vi "Single DM Control.vi"(7 "Calling VI Ref":refnum<vi>) -> ()   [LabVIEW 2016]
uses:
  Controls/Pixel Scan Parameters.ctl
  Controls/MirrorModes.ctl
  <vilib>/Utility/miscctls.llb/LVPointTypeDef.ctl
  Hardware Configuration/Hardware Configuration Controls/Standard Action.ctl
  <vilib>/Analysis/baseanly.llb/Mean (DBL).vi
  <vilib>/Utility/file.llb/Write Delimited Spreadsheet (DBL).vi
  <vilib>/Utility/file.llb/Read Delimited Spreadsheet (DBL).vi
  <vilib>/Analysis/NI_AALBase.lvlib
panel:
  in  "Load Control Matrix":bool
  in  "Bias Level":dbl format="%#_13g"
  in  "Load Flat":bool
  in  "Apply Zero":bool
  in  "Load V Map":bool
  in  "Save V Map":bool
  in  "Apply Flat":bool
  in  "Center Bias":bool
  in  "Quit":bool
  in  "Mirror Tab":enum32{"Mirror Modes", "Scan Pixels", "Poke"}(tab)
  in  "Clear Modes":bool
  in  "Mirror Modes":T1
  in  "Load Modes":bool
  in  "Save Modes":bool
  in  "Scan Modes":bool
  in  "Pixel Scan Save Path":path
  in  "Save Data":bool
  in  "Pixel Scan Parameters":T2={"Scan Start Pixel"=1, "Scan End Pixel"=1, "Pixel Start Value (-1 to 1)"=-0.5, "Pixel End Value (-1 to 1)"=0.5, "Number of Steps"=0.1}
  in  "Start Pixel Scan":bool
  in  "Poke Amount":dbl=1.0
  in  "Pixel No.":i32=1
  in  "Poke":bool
  in  "Poke Unit":T3(radio)
  out "Pixel Map (-1 to 1)":dbl[][](graph)
  # "Mode"
  # "Amount (nm)"
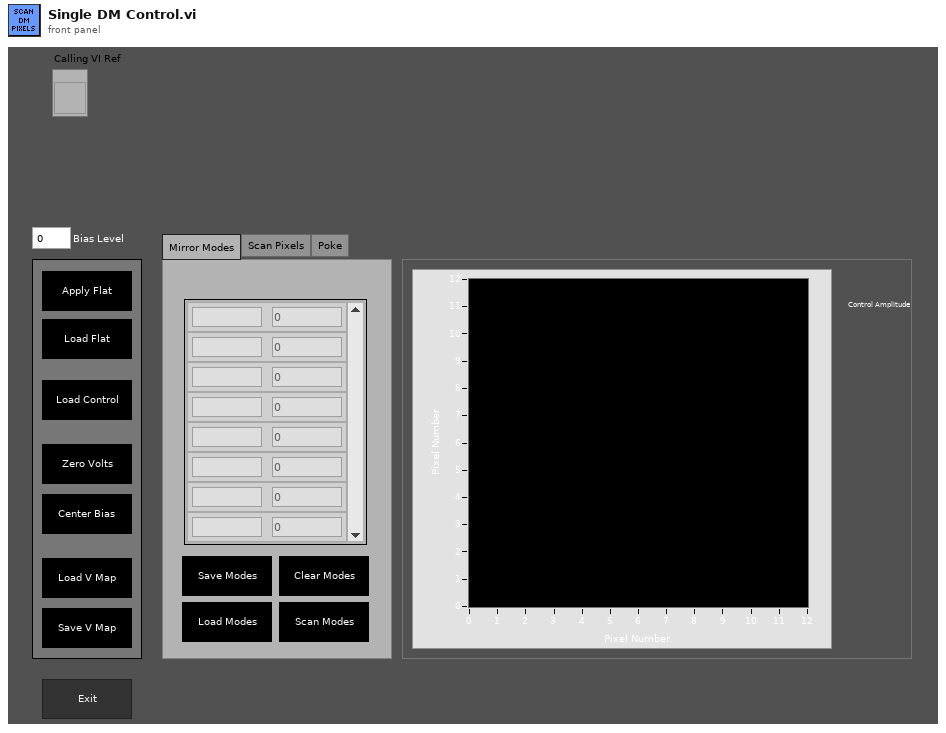
[diagram p1: front panel]
types:
  T1 = typedef "MirrorModes.ctl" = cluster{"Mode":string, "Amplitude":dbl}[]
  T2 = typedef "Pixel Scan Parameters.ctl" = cluster{"Scan Start Pixel":i32, "Scan End Pixel":i32, "Pixel Start Value (-1 to 1)":dbl, "Pixel End Value (-1 to 1)":dbl, "Number of Steps":dbl}
  T3 = enum32{"Voltage (V)", "Control Parameter [-1, 1]", "Approx. Distance (nm)"}
  T4 = enum16{"Always On", "Always Off", "Off While Running"}
  T5 = typedef "LVPointTypeDef.ctl" = cluster{"Horizontal":i16, "Vertical":i16}
  T6 = typedef "LVRectTypeDef.ctl" = cluster{"Left":i16, "Top":i16, "Right":i16, "Bottom":i16}
  T7 = typedef "LVBoundsTypeDef.ctl" = cluster{"Width":u32, "Height":u32}
  T8 = typedef "Standard Action.ctl" = enum16{"Read", "Write"}
  T9 = enum16{"Start Scan", "Reset Counter", "Write DM", "Get Image", "Update Count", "Exit"}
  T10 = enum32{"Invalid", "Standard", "Closed", "Hidden", "Minimized", "Maximized"}
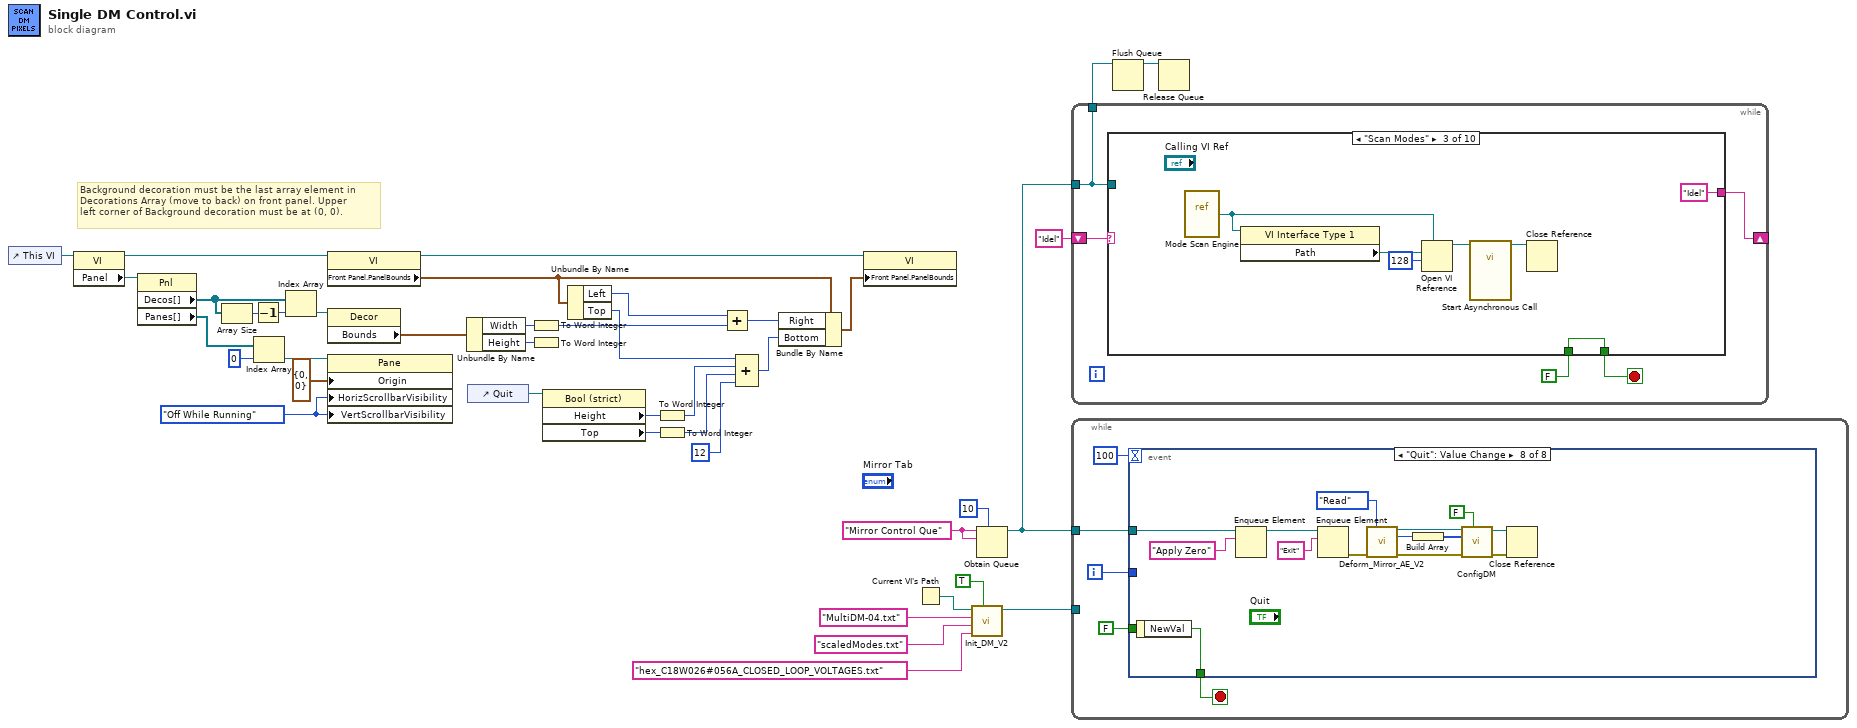
[diagram p0: block diagram]
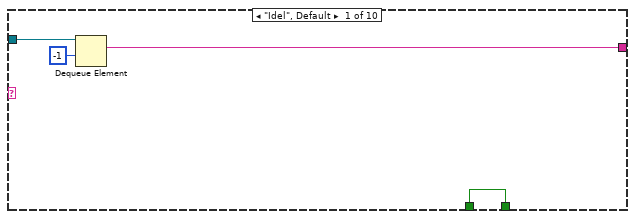
[diagram p2: hidden frame]
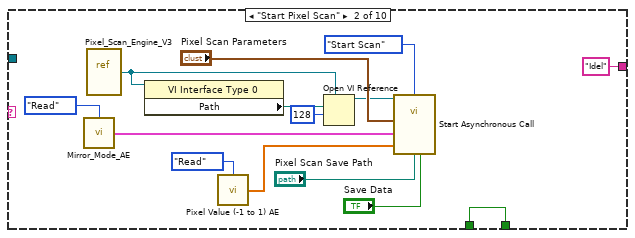
[diagram p3: hidden frame]
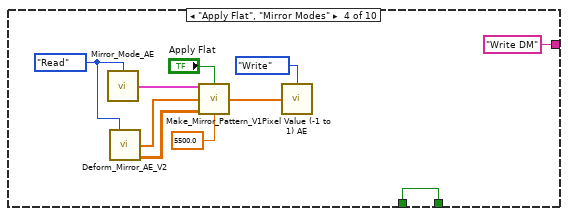
[diagram p4: hidden frame]
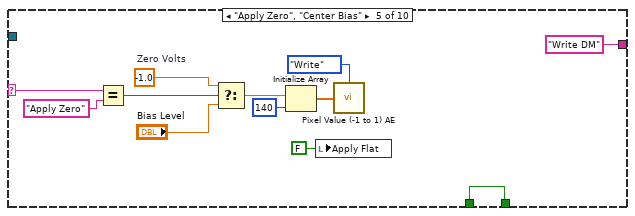
[diagram p5: hidden frame]
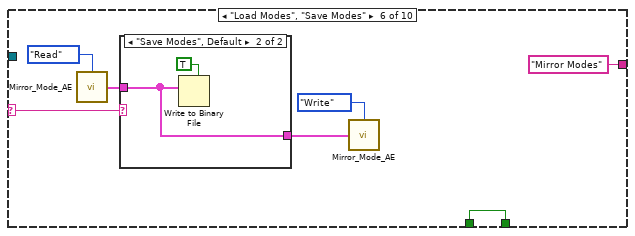
[diagram p6: hidden frame]
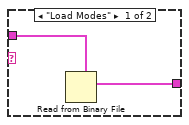
[diagram p7: hidden frame]
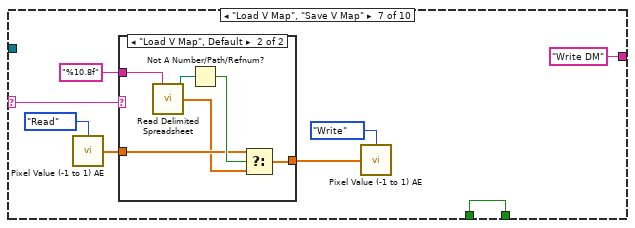
[diagram p8: hidden frame]
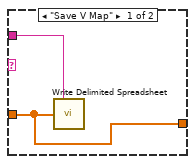
[diagram p9: hidden frame]
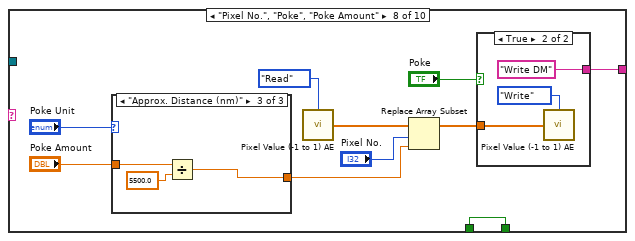
[diagram p10: hidden frame]
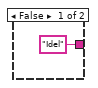
[diagram p11: hidden frame]
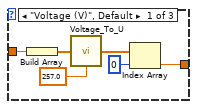
[diagram p12: hidden frame]
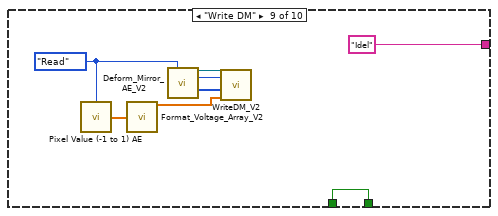
[diagram p14: hidden frame]
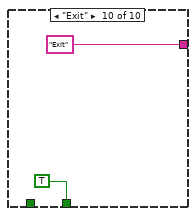
[diagram p15: hidden frame]
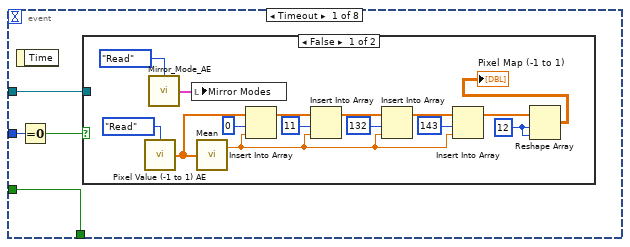
[diagram p16: hidden frame]
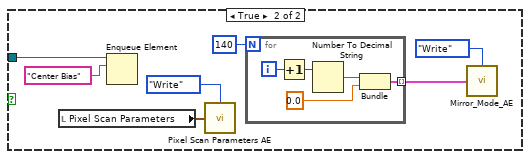
[diagram p17: hidden frame]
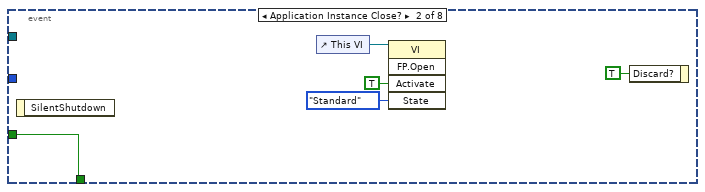
[diagram p18: hidden frame]
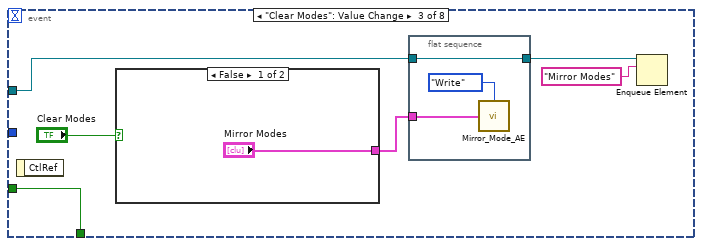
[diagram p19: hidden frame]
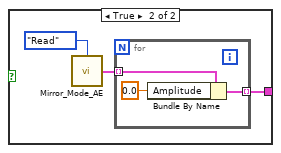
[diagram p20: hidden frame]
diagram:
  w12 = T4."Off While Running" ("Vertical Scrollbar Visibility")
  w41 = "Mirror Control Que" ("name (unnamed)")
  # "Background decoration must be the last array element in\nDecorations Array (move to back) on front panel. Upper\nleft corner of Background decoration must be at (0, 0)."
  n1 = control-ref of="This VI"() -> (w5:refnum<vi>)
  n2 = property class="VI"(reference=w5) -> (reference out=w13:refnum<vi>, "Panel"=w6:refnum<vi>)  [unwired: 1 in, 1 out]
  n3 = property class="Pnl"(reference=w6) -> ("Decos[]"=w4:refnum<vi>[], "Panes[]"=w9:refnum<vi>[])  [unwired: 1 in, 2 out]
  n4 = Array Size(array=w4) -> (size(s)=w2:i32)
  n5 = Decrement(x=w2) -> (x-1=w3:i32)
  n6 = Index Array(array=w9, index=0) -> (element=w8:refnum<vi>)
  n7 = Index Array(array=w4, index=w3) -> (element=w11:refnum<vi>)
  n8 = property class="VI"(reference=w13) -> (reference out=w15:refnum<vi>, "Front Panel.PanelBounds"=w16:T6)  [unwired: 1 in, 1 out]
  n9 = property class="Decor"(reference=w11) -> ("Bounds"=w14:T7)  [unwired: 1 in, 2 out]
  n10 = property class="Pane"(reference=w8, "Origin"=T5 {"Horizontal"=0, "Vertical"=0}, "HorizScrollbarVisibility"=w12, "VertScrollbarVisibility"=w12) -> ()  [unwired: 1 in, 2 out]
  n11 = Unbundle By Name(w14) -> ("Width"=w19:u32, "Height"=w22:u32)
  n12 = control-ref of="Quit"() -> (w1:refnum<vi>)
  n13 = To Word Integer(number=w19) -> (16bit integer=w21:i16)
  n14 = To Word Integer(number=w22) -> ()  [unwired: 1 out]
  n15 = property class="Bool (strict)"(reference=w1) -> ("Height"=w24:u32, "Top"=w25:i32)  [unwired: 1 in, 2 out]
  n16 = Unbundle By Name(w16) -> ("Left"=w18:i16, "Top"=w29:i16)
  n17 = To Word Integer(number=w24) -> (16bit integer=w27:i16)
  n18 = To Word Integer(number=w25) -> (16bit integer=w28:i16)
  n19 = Add(x=w18, y=w21) -> (x+y=w20:i16)
  n20 = Compound Arithmetic op=ADD(w29, w27, w28, i16 12 ("y")) -> (w23:i16)
  n21 = Bundle By Name(cluster=w16, "Right"=w20, "Bottom"=w23) -> (w17:T6)
  n22 = property class="VI"(reference=w15, "Front Panel.PanelBounds"=w17) -> ()  [unwired: 1 in, 2 out]
  n23 = Current VI's Path() -> (path=w33:path)
  n24 = call "Init_DM_V2.vi"("BM Flat"=TRUE, "BM Flat File"="hex_C18W026#056A_CLOSED_LOOP_VOLTAGES.txt" ("name or relative path"), "Mirror Modes File"="scaledModes.txt" ("name or relative path"), "DM Mapping File"="MultiDM-04.txt" ("name or relative path"), "Base File Path"=w33) -> ("reference out"=w39:refnum<k7>)  [unwired: 6 in]
  n25 = Obtain Queue(max queue size (-1, unlimited)=10, name (unnamed)=w41, element data type=w41) -> (queue out=w35:refnum<queue>)  [unwired: 2 in, 2 out]
  n26 = while {
    tunnel: w35 -> [w42]
    shift-right: [w46] -> _
    shift-left: "Idel" ("name (unnamed)") -> [w45]
    tunnel: [w42] -> w38
    stop <- w44 stop-if-true
    n27 = case shown="\"Scan Modes\"" w45 {
      selector: w45 -> [_ _ _ _ w88 w96 w111 _ _ _]
      tunnel: w42 -> [w50 _ _ _ _ _ _ _ _ _]
      tunnel: [w48 "Idel" ("name (unnamed)") "Idel" ("name (unnamed)") "Write DM" ("name (unnamed)") "Write DM" ("name (unnamed)") "Mirror Modes" ("name (unnamed)") "Write DM" ("name (unnamed)") w122 "Idel" ("name (unnamed)") "Exit" ("name (unnamed)")] -> w46
      tunnel: [w47 w64 w71 w80 w93 w100 w112 w130 w152 TRUE] -> w44
      tunnel: FALSE -> [w47 w64 w71 w80 w93 w100 w112 w130 w152 _]
      frame "Idel", Default {
        n28 = Dequeue Element(queue=w50, timeout in ms (-1)=-1) -> (element=w48:string)  [unwired: 1 in, 3 out]
      }
      frame "Start Pixel Scan" {
        n29 = call "Mirror_Mode_AE.vi"("Action"=Standard_Action."Read") -> ("Mirror Modes Out"=w51:T1)  [unwired: 14 in]
        n30 = vi-ref "Pixel_Scan_Engine_V3.vi"() -> (w55:refnum<vi>)
        n31 = property class="VI Interface Type 0"(reference=w55) -> ("Path"=w53:path)  [unwired: 1 in, 2 out]
        n32 = call "Pixel Value (-1 to 1) AE.vi"("Action"=Standard_Action."Read") -> ("Pixel Value (-1 to 1) Out"=w62:dbl[])  [unwired: 14 in]
        n33 = Open VI Reference(type specifier VI Refnum (for type only)=w55, vi path=w53, options=128) -> (vi reference=w56:refnum<vi>)  [unwired: 3 in, 1 out]
        n34 = call-by-ref "Start Asynchronous Call"(reference=w56, "Pixel Scan Parameters In"="Pixel Scan Parameters", "Action"=T9."Start Scan", "Initial Mirror Modes"=w51, "Initial Pixel Values (-1 to 1)"=w62, "Base Save Path"="Pixel Scan Save Path", "Save Data"="Save Data") -> ()  [unwired: 11 in, 2 out]
      }
      frame "Scan Modes" {
        n35 = vi-ref "Mode Scan Engine.vi"() -> (w65:refnum<vi>)
        n36 = property class="VI Interface Type 1"(reference=w65) -> ("Path"=w66:path)  [unwired: 1 in, 2 out]
        n37 = Open VI Reference(type specifier VI Refnum (for type only)=w65, vi path=w66, options=128) -> (vi reference=w68:refnum<vi>)  [unwired: 3 in, 1 out]
        n38 = call-by-ref "Start Asynchronous Call"(reference=w68) -> (reference out=w69:refnum<vi>)  [unwired: 17 in, 1 out]
        n39 = Close Reference(reference=w69) -> ()  [unwired: 1 in, 1 out]
      }
      frame "Apply Flat", "Mirror Modes" {
        w74 = Standard_Action."Read" ("Action")
        n40 = call "Mirror_Mode_AE.vi"("Action"=w74) -> ("Mirror Modes Out"=w77:T1)  [unwired: 14 in]
        n41 = call "Deform_Mirror_AE_V2.vi"("Action"=w74) -> ("Flat Files Out"=w78:dbl[], "Mode Matrix Out"=w79:dbl[][])  [unwired: 10 in, 3 out]
        n42 = call "Make_Mirror_Pattern_V1.vi"("Mirror Modes In"=w77, "Flat On?"="Apply Flat", "Flat File In"=w78, "Mirror Modes Array"=w79, "Amplitude Scale Factor"=5500.0) -> ("Pixel Value U (-1 to 1)"=w76:dbl[])  [unwired: 10 in]
        n43 = call "Pixel Value (-1 to 1) AE.vi"("Action"=Standard_Action."Write", "Pixel Value (-1 to 1)"=w76) -> ()  [unwired: 13 in, 1 out]
      }
      frame "Apply Zero", "Center Bias" {
        w84 = -1.0  # Zero Volts
        n44 = Equal?(x=w88, y="Apply Zero") -> (x = y?=w87:bool)
        n45 = Select(t=w84, s=w87, f="Bias Level") -> (s? t:f=w85:dbl)
        n46 = Initialize Array(w85, 140 ("dimension size")) -> (w91:dbl[])
        n47 = local write "Apply Flat"(FALSE ("Apply Flat")) -> ()
        n48 = call "Pixel Value (-1 to 1) AE.vi"("Action"=Standard_Action."Write", "Pixel Value (-1 to 1)"=w91) -> ()  [unwired: 13 in, 1 out]
      }
      frame "Load Modes", "Save Modes" {
        n49 = call "Mirror_Mode_AE.vi"("Action"=Standard_Action."Read") -> ("Mirror Modes Out"=w95:T1)  [unwired: 14 in]
        n50 = case shown="\"Save Modes\", Default" w96 {
          tunnel: w95 -> [w102 w103]
          tunnel: [w101 w103] -> w94
          frame "Load Modes" {
            n51 = Read from Binary File(5:w102) -> (2:w101:T1)  [unwired: 5 in, 3 out]
          }
          frame "Save Modes", Default {
            n52 = Write to Binary File(data=w103, 5:TRUE ("prepend array or string size? (T)")) -> ()  [unwired: 4 in, 3 out]
          }
        }
        n53 = call "Mirror_Mode_AE.vi"("Action"=Standard_Action."Write", "Mirror Modes In"=w94) -> ()  [unwired: 13 in, 1 out]
      }
      frame "Load V Map", "Save V Map" {
        n54 = call "Pixel Value (-1 to 1) AE.vi"("Action"=Standard_Action."Read") -> ("Pixel Value (-1 to 1) Out"=w109:dbl[])  [unwired: 14 in]
        n55 = case shown="\"Load V Map\", Default" w111 {
          tunnel: w109 -> [w113 w117]
          tunnel: "%10.8f" -> [w114 w120]
          tunnel: [w113 w115] -> w105
          frame "Save V Map" {
            n56 = call-poly <vilib>:"Write Delimited Spreadsheet.vi"("format (%.3f)"=w114, "1D data"=w113) -> ()  [unwired: 12 in, 2 out]
          }
          frame "Load V Map", Default {
            n57 = call-poly <vilib>:"Read Delimited Spreadsheet.vi"("format (%.3f)"=w120) -> ("new file path (Not A Path if cancelled)"=w119:path, "first row"=w116:dbl[])  [unwired: 9 in, 4 out]
            n58 = Not A Number/Path/Refnum?(number/path/refnum=w119) -> (NaN/Path/Refnum?=w118:bool)
            n59 = Select(t=w117, s=w118, f=w116) -> (s? t:f=w115:dbl[])
          }
        }
        n60 = call "Pixel Value (-1 to 1) AE.vi"("Action"=Standard_Action."Write", "Pixel Value (-1 to 1)"=w105) -> ()  [unwired: 13 in, 1 out]
      }
      frame "Pixel No.", "Poke", "Poke Amount" {
        n61 = case shown="\"Approx. Distance (nm)\"" "Poke Unit" {
          tunnel: "Poke Amount" -> [w139 w141 w144]
          tunnel: [w135 w141 w142] -> w128
          frame "Voltage (V)", Default {
            n62 = Build Array(w139) -> (w138:dbl[])
            n63 = call "Voltage_To_U.vi"("Voltages In (Volts)"=w138, "Mirror Max Voltage (Volts)"=257.0) -> ("Pixel Value (-1 to 1)"=w137:dbl[])  [unwired: 13 in]
            n64 = Index Array(array=w137, index=0) -> (element=w135:dbl)
          }
          frame "Control Parameter [-1, 1]" {
          }
          frame "Approx. Distance (nm)" {
            n65 = Divide(x=w144, y=5500.0) -> (x/y=w142:dbl)
          }
        }
        n66 = call "Pixel Value (-1 to 1) AE.vi"("Action"=Standard_Action."Read") -> ("Pixel Value (-1 to 1) Out"=w129:dbl[])  [unwired: 14 in]
        n67 = Replace Array Subset(array=w129, new element=w128, index="Pixel No.") -> (w123:dbl[])
        n68 = case shown="True" "Poke" {
          tunnel: w123 -> [_ w133]
          tunnel: ["Idel" ("name (unnamed)") "Write DM" ("name (unnamed)")] -> w122
          frame False {
          }
          frame True {
            n69 = call "Pixel Value (-1 to 1) AE.vi"("Action"=Standard_Action."Write", "Pixel Value (-1 to 1)"=w133) -> ()  [unwired: 13 in, 1 out]
          }
        }
      }
      frame "Write DM" {
        w150 = Standard_Action."Read" ("Action")
        n70 = call "Pixel Value (-1 to 1) AE.vi"("Action"=w150) -> ("Pixel Value (-1 to 1) Out"=w149:dbl[])  [unwired: 14 in]
        n71 = call "Format_Voltage_Array_V2.vi"("Pixel Level (-1 to 1)"=w149) -> ("Voltage Array (Volts)"=w145:dbl[])  [unwired: 13 in, 1 out]
        n72 = call "Deform_Mirror_AE_V2.vi"("Action"=w150) -> ("Refnum Out"=w148:refnum<k7>, "IDs Out"=w147:i32, "Multi Map Data Out"=w146:i32[])  [unwired: 10 in, 2 out]
        n73 = call "WriteDM_V2.vi"("reference in"=w148, "nDevId"=w147, "MultiDM  Mapping"=w146, "Voltage Array in"=w145) -> ()  [unwired: 2 in, 2 out]
      }
      frame "Exit" {
      }
    }
  }
  n74 = while {
    tunnel: w35 -> [w155]
    tunnel: w39 -> [_]
    i -> [w156]
    stop <- w159 stop-if-true
    n75 = event shown="[7] \"Quit\": Value Change" {
      selector: _ -> [_ _ _ _ _ _ _ _]
      dyn-events: _ -> [_ _ _ _ _ _ _ _]
      timeout: 100 -> [_ _ _ _ _ _ _ _]
      tunnel: [w163 w194 w201 w215 w221 w240 w254 w276] -> w159
      tunnel: FALSE -> [w163 w194 w201 w215 w221 w240 w254 _]
      tunnel: w156 -> [w162 _ _ _ _ _ _ _]
      tunnel: w155 -> [w160 _ w200 w214 _ _ _ w274]
      event Timeout {
        n76 = event-data() -> ()  [unwired: 1 in, 1 out]
        n77 = Equal To 0?(x=w162) -> (x = 0?=w161:bool)
        n78 = case shown="False" w161 {
          tunnel: w160 -> [_ w185]
          frame False {
            w177 = 12 ("dimension size")
            n79 = call "Pixel Value (-1 to 1) AE.vi"("Action"=Standard_Action."Read") -> ("Pixel Value (-1 to 1) Out"=w178:dbl[])  [unwired: 14 in]
            n80 = call "Mirror_Mode_AE.vi"("Action"=Standard_Action."Read") -> ("Mirror Modes Out"=w165:T1)  [unwired: 14 in]
            n81 = local write "Mirror Modes"(w165) -> ()
            n82 = call-poly <vilib>:"Mean.vi"("X"=w178) -> ("mean"=w175:dbl)  [unwired: 1 out]
            n83 = Insert Into Array(array=w178, index=0, new element=w175) -> (w170:dbl[])
            n84 = Insert Into Array(array=w170, index=11, new element=w175) -> (w172:dbl[])
            n85 = Insert Into Array(array=w172, index=132, new element=w175) -> (w174:dbl[])
            n86 = Insert Into Array(array=w174, index=143, new element=w175) -> (w167:dbl[])
            n87 = Reshape Array(w167, w177, w177) -> (→"Pixel Map (-1 to 1)":dbl[][])
          }
          frame True {
            n88 = local read "Pixel Scan Parameters"() -> (w182:T2)
            n89 = Enqueue Element(queue=w185, element="Center Bias") -> ()  [unwired: 2 in, 3 out]
            n90 = call "Pixel Scan Parameters AE.vi"("Action"=enum16{"Write", "Read"}."Write", "Pixel Scan Parameters"=w182) -> ()  [unwired: 13 in, 1 out]
            n91 = for {
              N: 140 -> [_]
              tunnel: [w186] -> w179 mode=indexing
              i -> [w190]
              n92 = Increment(x=w190) -> (x+1=w189:i32)
              n93 = Number To Decimal String(number=w189) -> (decimal integer string=w188:string)  [unwired: 1 in]
              n94 = Bundle(w188, 0.0) -> (w186:cluster{string, dbl})  [unwired: 1 in]
            }
            n95 = call "Mirror_Mode_AE.vi"("Action"=Standard_Action."Write", "Mirror Modes In"=w179) -> ()  [unwired: 13 in, 1 out]
          }
        }
      }
      event Application Instance Close? {
        n96 = event-data() -> ()  [unwired: 1 in, 1 out]
        n97 = control-ref of="This VI"() -> (w191:refnum<vi>)
        n98 = invoke class="VI" method="FP.Open"(reference=w191, "Activate"=TRUE ("Activate?"), "State"=T10."Standard") -> ()  [unwired: 2 in, 5 out]
        n99 = event-data("Discard?"=TRUE) -> ()  [unwired: 1 in, 1 out]
      }
      event "Clear Modes": Value Change {
        n100 = event-data() -> ()  [unwired: 1 in, 1 out]
        n101 = case shown="False" "Clear Modes" {
          tunnel: ["Mirror Modes" w203] -> w196
          frame False {
          }
          frame True {
            n102 = call "Mirror_Mode_AE.vi"("Action"=Standard_Action."Read") -> ("Mirror Modes Out"=w205:T1)  [unwired: 14 in]
            n103 = for {
              tunnel: w205 -> [w208] mode=indexing
              tunnel: [w206] -> w203 mode=indexing
              n104 = Bundle By Name(cluster=w208, "Amplitude"=0.0) -> (w206:cluster{"Mode":string, "Amplitude":dbl})
            }
          }
        }
        n105 = flat-sequence {
          tunnel: w196 -> [w210]
          tunnel: w200 -> [w209]
          tunnel: [w209] -> w198
          frame #0 {
            n106 = call "Mirror_Mode_AE.vi"("Action"=Standard_Action."Write", "Mirror Modes In"=w210) -> ()  [unwired: 13 in, 1 out]
          }
        }
        n107 = Enqueue Element(queue=w198, element="Mirror Modes") -> ()  [unwired: 2 in, 3 out]
      }
      event "Start Pixel Scan", "Apply Flat", "Center Bias", "Apply Zero", "Save V Map", "Save Modes", "Load Modes", "Load V Map", "Scan Modes", "Poke", "Pixel No.", "Poke Amount": Value Change {
        n108 = event-data() -> ("CtlRef"=w213:refnum<vi>)  [unwired: 1 in, 2 out]
        n109 = property class="Ctl"(reference=w213) -> ("Label.Text"=w212:string)  [unwired: 1 in, 2 out]
        n110 = Enqueue Element(queue=w214, element=w212) -> ()  [unwired: 2 in, 3 out]
      }
      event "Load Flat": Value Change {
        n111 = event-data() -> ()  [unwired: 1 in, 1 out]
        n112 = call-poly <vilib>:"Read Delimited Spreadsheet.vi"("format (%.3f)"="%10.8f") -> ("new file path (Not A Path if cancelled)"=w217:path, "first row"=w216:dbl[])  [unwired: 9 in, 4 out]
        n113 = Not A Number/Path/Refnum?(number/path/refnum=w217) -> (NaN/Path/Refnum?=w220:bool)
        n114 = case shown="False" w220 {
          tunnel: w216 -> [w234 _]
          tunnel: "Load Flat" -> [_ _]
          frame False {
            n115 = In Range and Coerce(upper limit=1.0, x=w234, lower limit=-1.0) -> (coerced(x)=w227:dbl[], In Range?=w231:bool[])
            n116 = call "Deform_Mirror_AE_V2.vi"("Action"=Standard_Action."Read") -> ("Refnum Out"=w223:refnum<k7>, "IDs Out"=w224:i32, "Multi Map Data Out"=w225:i32[], "Mode Matrix Out"=w226:dbl[][])  [unwired: 10 in, 1 out]
            n117 = Not(x=w231) -> (.not. x?=w230:bool[])
            n118 = Or Array Elements(Boolean array=w230) -> (logical OR=w222:bool)
            n119 = call "Deform_Mirror_AE_V2.vi"("Refnum In"=w223, "Action"=Standard_Action."Write", "IDs In"=w224, "Flat Files In"=w227, "Multi Map Data In"=w225, "Mode Matrix"=w226) -> ()  [unwired: 5 in, 5 out]
            n120 = case shown="True" w222 {
              frame False {
              }
              frame True {
                n121 = One Button Dialog(message="Flat File Out of Range [-1, 1]") -> ()  [unwired: 1 in, 1 out]
              }
            }
          }
          frame True {
          }
        }
      }
      event "Load Control Matrix": Value Change {
        n122 = event-data() -> ()  [unwired: 1 in, 1 out]
        n123 = call-poly <vilib>:"Read Delimited Spreadsheet.vi"("format (%.3f)"="%10.8f") -> ("new file path (Not A Path if cancelled)"=w239:path, "all rows"=w236:dbl[][])  [unwired: 9 in, 4 out]
        n124 = Not A Number/Path/Refnum?(number/path/refnum=w239) -> (NaN/Path/Refnum?=w237:bool)
        n125 = case shown="True" w237 {
          tunnel: w236 -> [_ w241]
          frame False {
          }
          frame True {
            n126 = call "Deform_Mirror_AE_V2.vi"("Action"=Standard_Action."Read") -> ("Refnum Out"=w244:refnum<k7>, "IDs Out"=w245:i32, "Flat Files Out"=w246:dbl[], "Multi Map Data Out"=w247:i32[])  [unwired: 10 in, 1 out]
            n127 = call "Deform_Mirror_AE_V2.vi"("Refnum In"=w244, "Action"=Standard_Action."Write", "IDs In"=w245, "Flat Files In"=w246, "Multi Map Data In"=w247, "Mode Matrix"=w241) -> ()  [unwired: 5 in, 5 out]
          }
        }
      }
      event "Poke Unit": Value Change {
        n128 = event-data() -> ("NewVal"=w252:T3)  [unwired: 1 in]
        n129 = local read "Pixel No."() -> (w248:i32)
        n130 = call "Pixel Value (-1 to 1) AE.vi"("Action"=Standard_Action."Read") -> ("Pixel Value (-1 to 1) Out"=w251:dbl[])  [unwired: 14 in]
        n131 = Index Array(array=w251, index=w248) -> (element=w250:dbl)
        n132 = case shown="\"Voltage (V)\", Default" w252 {
          tunnel: w250 -> [w259 w260 w263]
          tunnel: [w257 w260 w261] -> w249
          frame "Voltage (V)", Default {
            n133 = Build Array(w259) -> (w256:dbl[])
            n134 = call "Format_Voltage_Array_V2.vi"("Pixel Level (-1 to 1)"=w256) -> ("Voltage Array (Volts)"=w255:dbl[])  [unwired: 13 in, 1 out]
            n135 = Index Array(array=w255, index=0) -> (element=w257:dbl)
          }
          frame "Control Parameter [-1, 1]" {
          }
          frame "Approx. Distance (nm)" {
            n136 = Divide(x=w263, y=5500.0) -> (x/y=w261:dbl)
          }
        }
        n137 = local write "Poke Amount"(w249) -> ()
      }
      event "Quit": Value Change {
        n138 = event-data() -> ("NewVal"=w276:bool)  [unwired: 1 in]
        n139 = Enqueue Element(queue=w274, element="Apply Zero") -> (queue out=w273:refnum<queue>)  [unwired: 2 in, 2 out]
        n140 = Enqueue Element(queue=w273, element="Exit") -> (error out=w265:errorcluster)  [unwired: 2 in, 2 out]
        n141 = call "Deform_Mirror_AE_V2.vi"("Action"=Standard_Action."Read") -> ("Refnum Out"=w268:refnum<k7>, "IDs Out"=w269:i32)  [unwired: 10 in, 3 out]
        n142 = Build Array(w269) -> (w270:i32[])
        n143 = call "ConfigDM.vi"("High Voltage"=FALSE, "error in (no error)"=w265, "Dev IDs"=w270, "Automation Refnum in"=w268) -> ("error out"=w264:errorcluster, "Automation Refnum out"=w267:refnum<k7>)  [unwired: 6 in]
        n144 = Close Reference(reference=w267, error in (no error)=w264) -> ()  [unwired: 1 out]
      }
    }
  }
  n145 = Flush Queue(queue=w38) -> (queue out=w37:refnum<queue>)  [unwired: 1 in, 2 out]
  n146 = Release Queue(queue=w37) -> ()  [unwired: 2 in, 3 out]
